vi "VM - Close loose contexts.vi"(8 "error in":errorcluster, 11 "VC handles (all)":T1[](array[typedef])) -> (0 "error out":errorcluster, 1 "num of closed":i32)   [LabVIEW 2021]
doc: "This VI searches for loose contexts and closes them. This VI assumes that a context is loose if its creator VI is not in a state compatible with the context's lifetime specifier. Both the context's creator and its lifetime are defined when the context is created. Refer to the VI help for more details.\n\n::: CalcExpress Toolkit :::\nCopyright (c) 2000-2026 Konstantin Shifershteyn. All rights reserved."
uses:
  cetypes.llb/VarMan Variable Context Handle.ctl
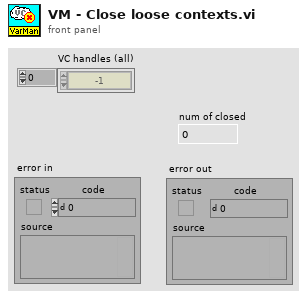
[diagram p1: front panel]
types:
  T1 = typedef "VarMan Variable Context Handle.ctl" = i32
  T2 = enum32{"Bad", "Idle", "Run top level", "Running"}
  T3 = typedef "VarMan Context Life Time.ctl" = enum32{"creator run top level", "creator running ", "creator in memory", "untill closed"}
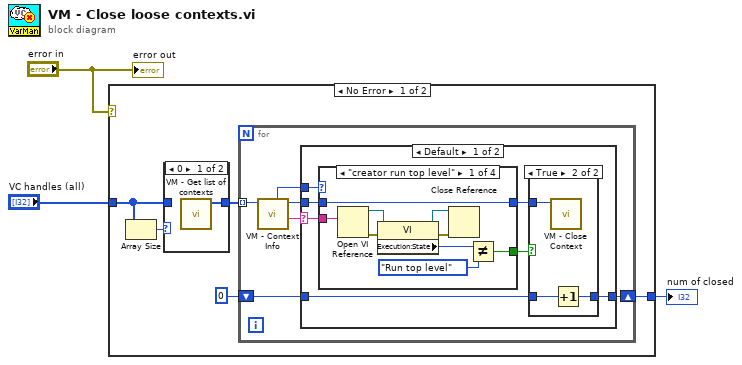
[diagram p0: block diagram]
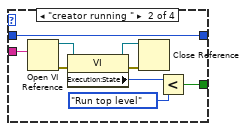
[diagram p4: hidden frame]
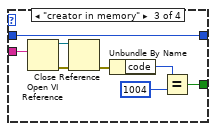
[diagram p5: hidden frame]
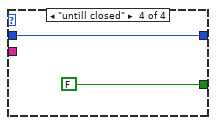
[diagram p6: hidden frame]
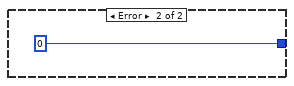
[diagram p8: hidden frame]
diagram:
  n1 = case shown="No Error" "error in" {
    tunnel: "VC handles (all)" -> [w6 _]
    tunnel: [w4 0] -> w1
    frame No Error {
      n2 = Array Size(array=w6) -> (size(s)=w7:i32)
      n3 = case shown="0" w7 {
        tunnel: [w9 w10] -> w8
        tunnel: w6 -> [_ w10]
        frame 0 {
          n4 = call "VM - Get list of contexts.vi"() -> ("array of VC handles"=w9:T1[])  [unwired: 7 in, 2 out]
        }
        frame 1, Default {
        }
      }
      n5 = for {
        tunnel: w8 -> [w16] mode=indexing
        shift-right: [w11] -> w4
        shift-left: 0 -> [w12]
        n6 = call "VM - Context Info.vi"("VC Handle"=w16) -> ("Creator"=w15:string, "dup VC Handle"=w13:T1, "context life time"=w14:T3)  [unwired: 6 in, 2 out]
        n7 = case shown="Default" w15 {
          selector: w15 -> [w22 _]
          tunnel: w14 -> [w23 _]
          tunnel: w13 -> [w21 _]
          tunnel: w12 -> [w18 w56]
          tunnel: [w17 w56] -> w11
          frame Default {
            n8 = case shown="\"creator run top level\"" w23 {
              tunnel: w22 -> [w36 w45 w53 _]
              tunnel: [w28 w37 w49 FALSE] -> w20
              tunnel: [w31 w40 w46 w54] -> w19
              tunnel: w21 -> [w31 w40 w46 w54]
              frame "creator run top level" {
                n9 = Open VI Reference(vi path=w36) -> (vi reference=w35:refnum<vi>, error out=w34:errorcluster)  [unwired: 5 in]
                n10 = property on="Property Node" class="VI"(reference=w35, error in=w34) -> (reference out=w32:refnum<vi>, error out=w33:errorcluster, "Execution:State"=w30:T2)
                n11 = Close Reference(reference=w32, error in (no error)=w33) -> ()  [unwired: 1 out]
                n12 = Not Equal?(x=w30, y=T2."Run top level" ("Execution:State")) -> (x != y?=w28:bool)
              }
              frame "creator running " {
                n13 = Open VI Reference(vi path=w45) -> (vi reference=w44:refnum<vi>, error out=w43:errorcluster)  [unwired: 5 in]
                n14 = property on="Property Node" class="VI"(reference=w44, error in=w43) -> (reference out=w41:refnum<vi>, error out=w42:errorcluster, "Execution:State"=w39:T2)
                n15 = Close Reference(reference=w41, error in (no error)=w42) -> ()  [unwired: 1 out]
                n16 = Less?(x=w39, y=T2."Run top level" ("Execution:State")) -> (x < y?=w37:bool)
              }
              frame "creator in memory" {
                n17 = Open VI Reference(vi path=w53) -> (vi reference=w51:refnum<vi>, error out=w52:errorcluster)  [unwired: 5 in]
                n18 = Close Reference(reference=w51, error in (no error)=w52) -> (error out=w50:errorcluster)
                n19 = Unbundle By Name(w50) -> ("code"=w48:i32)
                n20 = Equal?(x=w48, y=1004) -> (x = y?=w49:bool)
              }
              frame "untill closed" {
              }
            }
            n21 = case shown="True" w20 {
              tunnel: w19 -> [_ w27]
              tunnel: w18 -> [w24 w26]
              tunnel: [w24 w25] -> w17
              frame False {
              }
              frame True {
                n22 = call "VM - Close Context.vi"("VC Handle"=w27) -> ()  [unwired: 9 in, 2 out]
                n23 = Increment(x=w26) -> (x+1=w25:i32)
              }
            }
          }
          frame "" {
          }
        }
      }
    }
    frame Error {
    }
  }
  "num of closed" <- w1
  "error out" <- "error in"
